vi "temperature global.vi"() -> ()   [LabVIEW 2026]
panel:
  out "Temperature Global":dbl[](array[numeric])
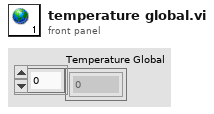
[diagram p1: front panel]
diagram:
